vi "add point to batch buffer.vi"(7 "channel tags":cluster{"key":string, "value":string}[](array[cluster]), 8 "Value":dbl, 9 "Time Stamp":timestamp, 10 "channel":string, 11 "batch buffer":refnum<data-value>) -> (0 "error out":errorcluster)   [LabVIEW 2020, in "nominal core steps.lvlib"]
doc: "In the provided buffer session, add data for a channel. Channels are uniquely identified by the combination of a name and optional tags.\n\nExamples:\nCall with \"name\", <no tags>; Call with \"name\", <no tags> => one channel\nCall with \"name\", <no tags>; Call with \"name\", tags: [sn: 123] => two channels\nCall with \"name\", tags: [sn: 123]; Call with \"name\", tags: [sn: 321] => two channels"
uses:
  nominal core steps.lvlib
  points buffer.ctl
  batch buffer.ctl
  single point.ctl
  channel uid.ctl
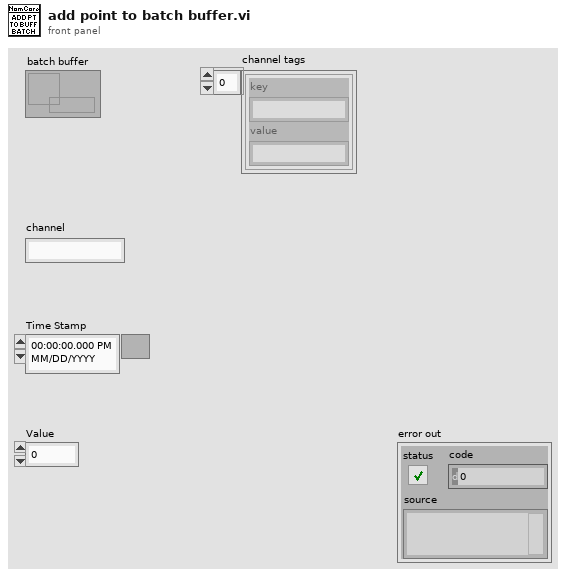
[diagram p1: front panel]
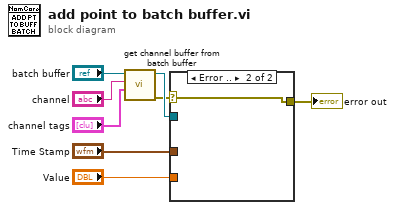
[diagram p0: block diagram]
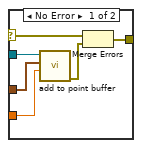
[diagram p2: hidden frame]
diagram:
  n1 = call "get channel buffer from batch buffer.vi"("channel tags"="channel tags", "channel"="channel", "batch buffer"="batch buffer") -> ("error out"=w1:errorcluster, "channel point buffer"=w3:refnum<data-value>)  [unwired: 7 in]
  n2 = case shown="Error .." w1 {
    selector: w1 -> [w9 w15]
    tunnel: "Time Stamp" -> [w14 _]
    tunnel: "Value" -> [w13 _]
    tunnel: w3 -> [w12 _]
    tunnel: [w10 w15] -> w2
    frame No Error {
      n3 = call "add to point buffer.vi"("value"=w13, "time"=w14, "point buffer"=w12) -> ("error out"=w11:errorcluster)  [unwired: 8 in]
      n4 = Merge Errors(w9, w11) -> (w10:errorcluster)
    }
    frame Error {
    }
  }
  "error out" <- w2
